vi "Write Sensor K-Values.vi"(10 "Sensor K-Values":void[](array[numeric]), 11 "LabjacksController in":refnum<class "LabjacksController.lvclass">) -> (3 "LabjacksController out":refnum<class "LabjacksController.lvclass">)   [LabVIEW 2025, in "LabjacksController.lvclass"]
uses:
  LabjacksController.lvclass
  LabjacksController.lvclass/LabjacksController.ctl
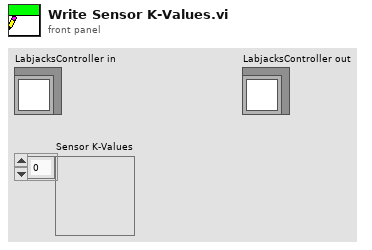
[diagram p1: front panel]
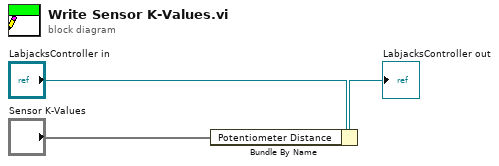
[diagram p0: block diagram]
diagram:
  n1 = Bundle By Name(cluster="LabjacksController in", "Potentiometer Distance"="Sensor K-Values") -> (→"LabjacksController out":refnum<class "LabjacksController.lvclass">)
